vi "KalmanFilterLatencyComp_ApplyPastGlobalMeas_FuncGroup.vi"(6 "VisionCorrectExtra":variant, 7 "F_Func":T2, 8 "VisionCorrect_Func":refnum<vi>, 9 "H_FuncExtra":variant, 10 "H_Func":T2, 11 "F_FuncExtra":variant) -> (0 "Error":errorcluster, 3 "KALMAN_FILTER_LATENCY_COMP_FUNC_GROUP":T1)   [LabVIEW 2019, in "Trajectory_Library.lvlib"]
doc: "Packs the individual function references and extra data into a cluster to pass to ApplyPastGlobalMeasurements. \n\nInputs:\n - F_Func -- \n - F_FuncExtra -- variant containing the extra data, if any, required by the F_Func\n - H_Func -- \n - H_FuncExtra -- variant containing the extra data, if any, required by the F_Func\n - VisionCorrect_Func -- \n - VisionCorrectExtra -- variant containing the extra data, if any, required by the VIsionCorrect_Func\n\nOutputs:\n - Comp_Func_Group -- Packed data cluster\n - Error -- If TRUE, an error occured."
uses:
  Trajectory_Library.lvlib
  TypeDef/CALLBACK_FUNC_TYPE.ctl
  TypeDef/KALMAN_FILTER_LATENCY_COMP_FUNC_GROUP.ctl
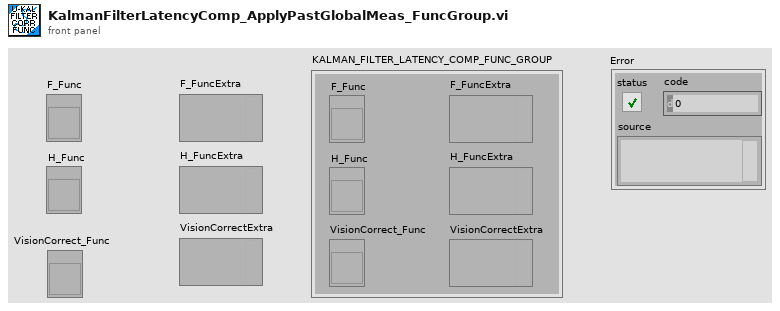
[diagram p1: front panel]
types:
  T1 = typedef "Trajectory_Library.lvlib/KALMAN_FILTER_LATENCY_COMP_FUNC_GROUP.ctl" = cluster{"F_Func":T2, "H_Func":T2, "F_FuncExtra":variant, "H_FuncExtra":variant, "VisionCorrectExtra":variant, "VisionCorrect_Func":refnum<vi>}
  T2 = typedef "Trajectory_Library.lvlib/CALLBACK_FUNC_TYPE.ctl" = refnum<vi>
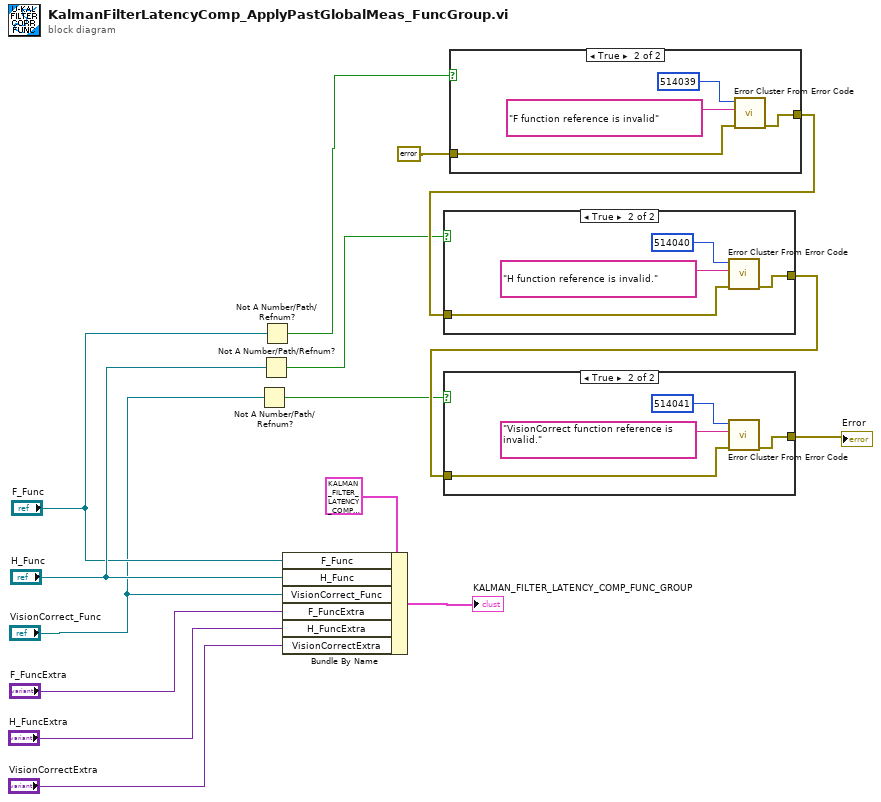
[diagram p0: block diagram]
diagram:
  n1 = Not A Number/Path/Refnum?(number/path/refnum="VisionCorrect_Func") -> (NaN/Path/Refnum?=w2:bool)
  n2 = Not A Number/Path/Refnum?(number/path/refnum="H_Func") -> (NaN/Path/Refnum?=w3:bool)
  n3 = Not A Number/Path/Refnum?(number/path/refnum="F_Func") -> (NaN/Path/Refnum?=w4:bool)
  n4 = Bundle By Name(cluster=T1 {"F_Func"=refnum, "H_Func"=refnum, "F_FuncExtra"=variant, "H_FuncExtra"=variant, "VisionCorrectExtra"=variant, "VisionCorrect_Func"=refnum} ("UNSCENTED_KALMAN_FILTER_FUNC_GROUP"), "F_Func"="F_Func", "H_Func"="H_Func", "VisionCorrect_Func"="VisionCorrect_Func", "F_FuncExtra"="F_FuncExtra", "H_FuncExtra"="H_FuncExtra", "VisionCorrectExtra"="VisionCorrectExtra") -> (→"KALMAN_FILTER_LATENCY_COMP_FUNC_GROUP":T1)
  n5 = case shown="True" w4 {
    tunnel: errorcluster {"status"=FALSE, "code"=0, "source"=""} ("error constant") -> [w16 w19]
    tunnel: [w16 w20] -> w6
    frame False {
    }
    frame True {
      n6 = call <vilib>:"Error Cluster From Error Code.vi"("error in (no error)"=w19, "error message (\"\")"="F function reference is invalid" ("error message (\"\")"), "error code (0)"=514039) -> ("error out"=w20:errorcluster)  [unwired: 6 in]
    }
  }
  n7 = case shown="True" w3 {
    tunnel: w6 -> [w21 w24]
    tunnel: [w21 w25] -> w5
    frame False {
    }
    frame True {
      n8 = call <vilib>:"Error Cluster From Error Code.vi"("error in (no error)"=w24, "error message (\"\")"="H function reference is invalid." ("error message (\"\")"), "error code (0)"=514040) -> ("error out"=w25:errorcluster)  [unwired: 6 in]
    }
  }
  n9 = case shown="True" w2 {
    tunnel: w5 -> [w26 w29]
    tunnel: [w26 w30] -> w1
    frame False {
    }
    frame True {
      n10 = call <vilib>:"Error Cluster From Error Code.vi"("error in (no error)"=w29, "error message (\"\")"="VisionCorrect function reference is invalid." ("error message (\"\")"), "error code (0)"=514041) -> ("error out"=w30:errorcluster)  [unwired: 6 in]
    }
  }
  "Error" <- w1
